vi "VIH HelpGen - Write HTML File - Menu - Subpalette Table.vi"(4 "Show Item Icons":bool, 5 "HTML Folder":path, 6 "Items":T1, 7 "Image Folder":path, 8 "error in":errorcluster, 9 "Table Templates":T2, 10 "HTML in":string, 11 "Menu Path":path) -> (0 "error out":errorcluster, 2 "HTML out":string)   [LabVIEW 2014]
doc: "::: VI Helpeks :::\nCopyright (c) 2000-2026 Konstantin Shifershteyn. All rights reserved."
uses:
  VIH HelpGen Typedef - Table Templates Cluster - Menu Help.ctl
  VIH HelpGen Typedef - Enum - Description Mode.ctl
panel:
  # "VI Helpeks\nCopyright (c) 2012-2026 Konstantin Shifershteyn"
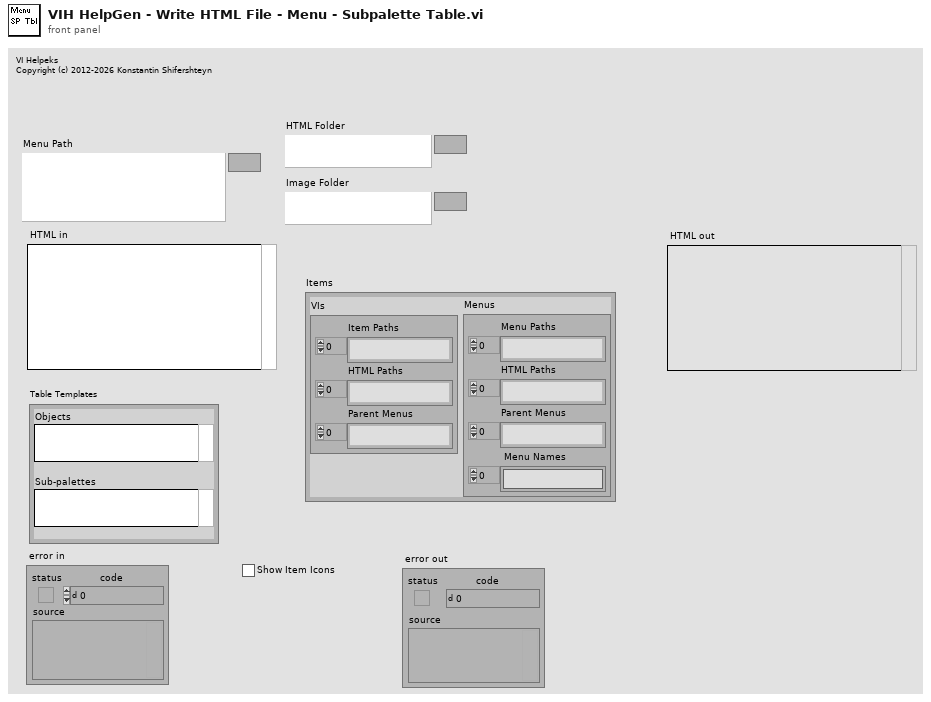
[diagram p1: front panel]
types:
  T1 = cluster{"VIs":cluster{"Item Paths":path[], "HTML Paths":path[], "Parent Menus":path[]}, "Menus":cluster{"Menu Paths":path[], "HTML Paths":path[], "Parent Menus":path[], " Menu Names":string[]}}
  T2 = typedef "VIH HelpGen Typedef - Table Templates Cluster - Menu Help.ctl" = cluster{"Objects":string, "Sub-palettes":string}
  T3 = typedef "VIH HelpGen Typedef - Palette - Item Info Cluster.ctl" = cluster{"Item Type":T4, "Item Name":string, "Item File":path, "Parent palette":path, "Not found":bool}
  T4 = typedef "VIH HelpGen Typedef - Palette - Item Type Enum.ctl" = enum32{"<Invalid>", "<unknown>", "VI", "Menu", "LV Func", "Express VI", "Poly VI", "CTL", "HTML"}
  T5 = cluster{"Menu Paths":path[], "HTML Paths":path[], "Parent Menus":path[], " Menu Names":string[]}
  T6 = typedef "VIH HelpGen Typedef - Enum - Description Mode.ctl" = enum16{"Default", "Description", "Description1", "Description2", "Custom", "None"}
  T7 = typedef "Palette Menu.lvlib/Palette Data.ctl" = cluster{"display name":string, "view format":T8, "palette width":i16, "items":T9, "256 color icon":picture, "B&W color icon":picture, "help information":T11, "palette description":string, "synchronize information":T12}
  T8 = typedef "Palette Menu.lvlib/View Format.ctl" = u16
  T9 = typedef "Palette Menu.lvlib/Items.ctl" = T10[]
  T10 = typedef "Palette Menu.lvlib/Item.ctl" = cluster{"item path":path, "library path (.lvlib)":path, "use default lvlib palette":bool, "short name":string, "place VI contents":bool, "hide synchronized item":bool, "reserve spot for synch item":bool, "configure when placing VI contents":bool}
  T11 = typedef "Palette Menu.lvlib/Help Info.ctl" = cluster{"help tag":string, "help file path ":path}
  T12 = typedef "Palette Menu.lvlib/Synchronize Info.ctl" = cluster{"synchronize with directory":bool, "synchronize directory path":path}
  T13 = typedef "imagedata.ctl" = cluster{"image type":i32, "image depth":i32, "image":u8[], "mask":u8[], "colors":u32[], "Rectangle":cluster{"left":i16, "top":i16, "right":i16, "bottom":i16}}
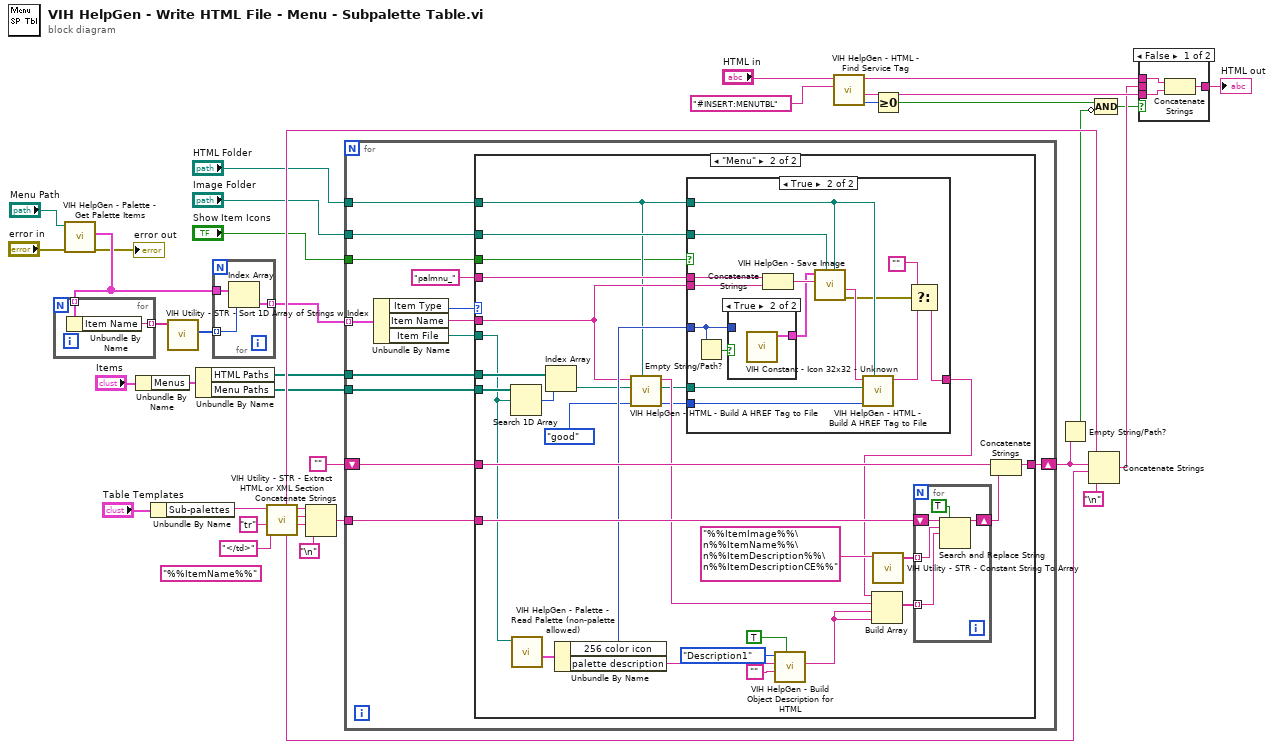
[diagram p0: block diagram]
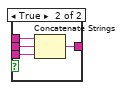
[diagram p2: hidden frame]
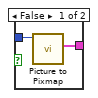
[diagram p5: hidden frame]
diagram:
  (unwired) "%%ItemName%%"
  n1 = call "VIH HelpGen - Palette - Get Palette Items.vi"("error in"="error in", "Palette Path"="Menu Path") -> ("error out"=→"error out":errorcluster, "Items Array"=w4:T3[])  [unwired: 7 in, 1 out]
  n2 = for {
    tunnel: [w40] -> w7 mode=indexing
    tunnel: w4 -> [w39] mode=indexing
    n3 = Unbundle By Name(w39) -> ("Item Name"=w40:string)
  }
  n4 = Unbundle By Name("Items") -> ("Menus"=w10:T5)
  n5 = Unbundle By Name("Table Templates") -> ("Sub-palettes"=w21:string)
  n6 = call "VIH Utility - STR - Sort 1D Array of Strings w Index.vi"("Array in"=w7) -> ("Index array"=w6:i32[])  [unwired: 7 in, 3 out]
  n7 = Unbundle By Name(w10) -> ("HTML Paths"=w18:path[], "Menu Paths"=w19:path[])
  n8 = for {
    tunnel: w4 -> [w43]
    tunnel: w6 -> [w42] mode=indexing
    tunnel: [w41] -> w5 mode=indexing
    n9 = Index Array(array=w43, index=w42) -> (element=w41:T3)
  }
  n10 = call "VIH Utility - STR - Extract HTML or XML Section.vi"("Contain (opt)"="</td>", "Section name"="tr", "HTML in"=w21) -> ("end"=w30:string, "body"=w31:string, "start"=w32:string, "after"=w24:string, "before"=w25:string)  [unwired: 4 in]
  n11 = Concatenate Strings(w32, w31, w30, "\n") -> (w27:string)
  n12 = for {
    tunnel: w5 -> [w56] mode=indexing
    shift-right: [w50] -> w16
    shift-left: "" -> [w51]
    tunnel: w27 -> [w54]
    tunnel: w19 -> [w49]
    tunnel: w18 -> [w48]
    tunnel: "HTML Folder" -> [w47]
    tunnel: "Image Folder" -> [w46]
    tunnel: "Show Item Icons" -> [w44]
    n13 = Unbundle By Name(w56) -> ("Item Type"=w55:T4, "Item Name"=w53:string, "Item File"=w52:path)
    n14 = case shown="\"Menu\"" w55 {
      tunnel: w54 -> [_ w83]
      tunnel: w53 -> [_ w73]
      tunnel: w52 -> [_ w59]
      tunnel: w51 -> [w57 w82]
      tunnel: [w57 w81] -> w50
      tunnel: w49 -> [_ w79]
      tunnel: w48 -> [_ w78]
      tunnel: w47 -> [_ w71]
      tunnel: w46 -> [_ w76]
      tunnel: "palmnu_" -> [_ w75]
      tunnel: w44 -> [_ w62]
      frame Default {
      }
      frame "Menu" {
        n15 = Search 1D Array(1D array=w79, element=w59) -> (index of element=w77:i32)  [unwired: 1 in]
        n16 = call "VIH HelpGen - Palette - Read Palette (non-palette allowed).vi"("Palette Path"=w59) -> ("palette data"=w60:T7)  [unwired: 8 in, 2 out]
        n17 = Index Array(array=w78, index=w77) -> (element=w70:path)
        n18 = Unbundle By Name(w60) -> ("256 color icon"=w74:picture, "palette description"=w66:string)
        n19 = call "VIH HelpGen - HTML - Build A HREF Tag to File.vi"("HTML Folder"=w71, "file status"=enum16{"unknown", "good", "bad"}."good", "Referenced HTML File"=w70, "Name"=w73) -> ("file status out"=w68:enum16{"unknown", "good", "bad"}, "dup Referenced HTML File"=w69:path, "HTML out"=w72:string)  [unwired: 5 in]
        n20 = case shown="True" w62 {
          tunnel: w76 -> [_ w100]
          tunnel: w75 -> [_ w99]
          tunnel: w74 -> [_ w88]
          tunnel: w73 -> [_ w98]
          tunnel: w71 -> [_ w97]
          tunnel: [_ w89] -> w61
          tunnel: w69 -> [_ w96]
          tunnel: w68 -> [_ w95]
          frame False {
          }
          frame True {
            n21 = Empty String/Path?(string/path=w88) -> (empty?=w87:bool)
            n22 = case shown="True" w87 {
              tunnel: [w103 w104] -> w93
              tunnel: w88 -> [w102 _]
              frame False {
                n23 = call <vilib>:"Picture to Pixmap.vi"("picture"=w102) -> ("image data"=w103:T13)  [unwired: 9 in, 1 out]
              }
              frame True {
                n24 = call "VIH Constant - Icon 32x32 - Unknown.vi"() -> ("image data"=w104:T13)  [unwired: 11 in]
              }
            }
            n25 = Concatenate Strings(w99, w98) -> (w101:string)
            n26 = call "VIH HelpGen - Save Image.vi"("HTML Folder"=w97, "Image Folder"=w100, "Image Filename"=w101, "image data"=w93) -> ("error out"=w91:errorcluster, "HTML tag"=w94:string)  [unwired: 5 in, 1 out]
            n27 = call "VIH HelpGen - HTML - Build A HREF Tag to File.vi"("HTML Folder"=w97, "file status"=w95, "Referenced HTML File"=w96, "Name"=w94) -> ("HTML out"=w90:string)  [unwired: 5 in, 2 out]
            n28 = Select(t="", s=w91, f=w90) -> (s? t:f=w89:string)
          }
        }
        n29 = call "VIH HelpGen - Build Object Description for HTML.vi"("Ena \"No Description\" message (F)"=TRUE, "Custom Description"="", "Default Description"=w66, "DscrMode"=VIH_HelpGen_Typedef_-_Enum_-_Description_Mode."Description1") -> ("Description HTML out"=w58:string)  [unwired: 6 in, 1 out]
        n30 = Build Array(w61, w72, w58, w58) -> (w84:string[])
        n31 = call "VIH Utility - STR - Constant String To Array.vi"("String in"="%%ItemImage%%\n%%ItemName%%\n%%ItemDescription%%\n%%ItemDescriptionCE%%") -> ("Array out"=w85:string[])  [unwired: 10 in]
        n32 = for {
          shift-right: [w108] -> w80
          shift-left: w83 -> [w109]
          tunnel: w85 -> [w106] mode=indexing
          tunnel: w84 -> [w105] mode=indexing
          n33 = Search and Replace String(replace all?=TRUE, input string=w109, search string=w106, replace string=w105) -> (result string=w108:string)  [unwired: 4 in, 3 out]
        }
        n34 = Concatenate Strings(w82, w80) -> (w81:string)
      }
    }
  }
  n35 = call "VIH HelpGen - HTML - Find Service Tag.vi"("Tag name"="#INSERT:MENUTBL", "HTML in"="HTML in") -> ("Offset out"=w15:i32, "After"=w36:string, "Before"=w37:string)  [unwired: 6 in, 1 out]
  n36 = Greater Or Equal To 0?(x=w15) -> (x >= 0?=w14:bool)
  n37 = Empty String/Path?(string/path=w16) -> (empty?=w13:bool)
  n38 = Concatenate Strings(w25, w16, w24, "\n") -> (w23:string)
  n39 = Compound Arithmetic op=AND(w14, invert w13) -> (w12:bool)
  n40 = case shown="False" w12 {
    tunnel: w23 -> [_ w116]
    tunnel: [w111 w115] -> w26
    tunnel: w37 -> [w112 w114]
    tunnel: w36 -> [w110 w113]
    frame False {
      n41 = Concatenate Strings(w112, w110) -> (w111:string)
    }
    frame True {
      n42 = Concatenate Strings(w114, w116, w113) -> (w115:string)
    }
  }
  "HTML out" <- w26
